vi "Assert Equal Type_Variant.vi"(4 "Execution time (s)":dbl=-1.0, 5 "Assert Only? (F)":bool, 6 "error code (1)":i32=1, 7 "Label":string, 8 "error in (no error)":errorcluster, 9 "Register with caller test (F)":bool, 10 "Actual":variant, 11 "Expected":variant) -> (0 "error out":errorcluster, 2 "Properties.Assert":refnum<class "Properties.Assert.lvclass">)   [LabVIEW 2013, in "Caraya.lvlib" / "Assert.lvclass"]
doc: "Generates an error if the input condition is not met.\n\nThis method compares the value of the inputs, irrespective of the type representation.\nAsserts TRUE if input values are equal.\nAsserts FALSE otherwise.\n\nex: Two integer inputs of equal value but of different type representation (U8 and I32) will assert TRUE."
uses:
  Assert.lvclass
  Properties.Assert/Properties.Assert.lvclass
  Properties/Properties.lvclass
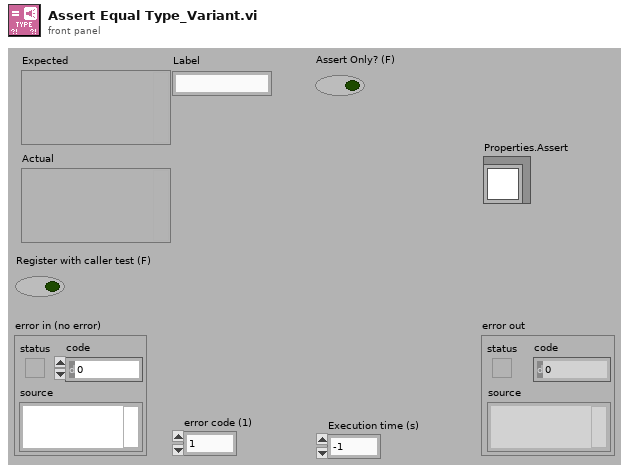
[diagram p1: front panel]
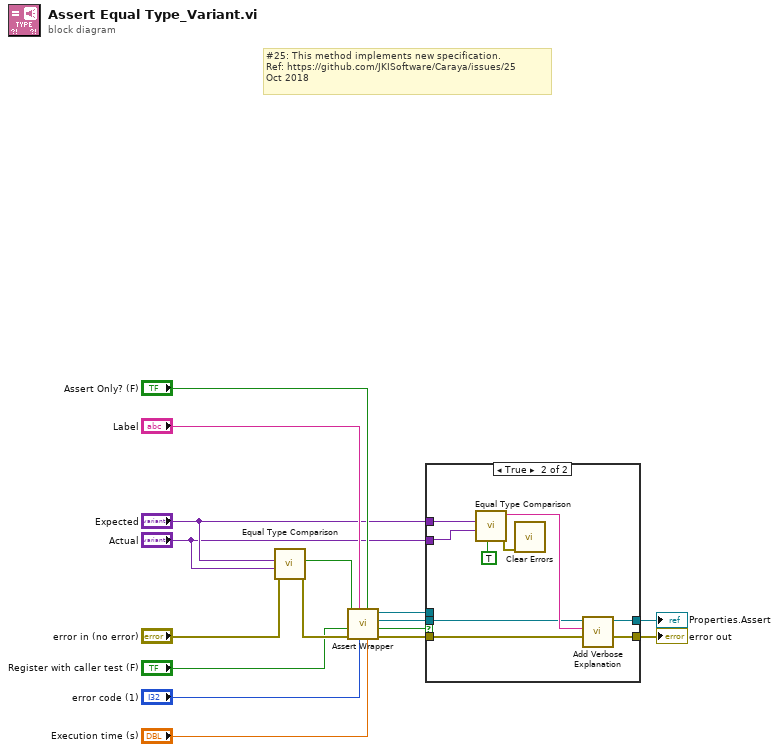
[diagram p0: block diagram]
diagram:
  # "#25: This method implements new specification.\nRef: https://github.com/JKISoftware/Caraya/issues/25\nOct 2018"
  n1 = call "Equal Type Comparison.vi"("error in (no error)"="error in (no error)", "Actual"="Actual", "Expected"="Expected") -> ("error out"=w13:errorcluster, "Equal Types?"=w12:bool)  [unwired: 6 in, 1 out]
  n2 = call "Assert Wrapper.vi"("Execution time (s)"="Execution time (s)", "Assert Only? (F)"="Assert Only? (F)", "error code (1)"="error code (1)", "Label"="Label", "error in (no error)"=w13, "Register with caller test (F)"="Register with caller test (F)", "Assert?"=w12) -> ("error out"=w9:errorcluster, "Verbose"=w5:bool, "Properties.Assert"=w2:refnum<class "Properties.Assert.lvclass">, "Assert out"=w3:refnum<class "Assert.lvclass">)  [unwired: 1 in]
  n3 = case shown="True" w5 {
    tunnel: [w18 w22] -> w10
    tunnel: w3 -> [_ _]
    tunnel: w9 -> [w18 w21]
    tunnel: "Expected" -> [_ w27]
    tunnel: "Actual" -> [_ w26]
    tunnel: w2 -> [w17 w20]
    tunnel: [w17 w19] -> w1
    frame False {
    }
    frame True {
      n4 = call "Equal Type Comparison.vi"("verbose? (F)"=TRUE, "Actual"=w26, "Expected"=w27) -> ("error out"=w24:errorcluster, "Verbose output"=w23:string)  [unwired: 6 in, 1 out]
      n5 = call <vilib>:"Clear Errors.vi"("error in (no error)"=w24) -> ()  [unwired: 6 in, 1 out]
      n6 = call "Add Verbose Explanation.vi"("error in (no error)"=w21, "Verbose Explanation"=w23, "Properties"=w20) -> ("error out"=w22:errorcluster, "Properties"=w19:refnum<class "Properties.Assert.lvclass">)  [unwired: 7 in]
    }
  }
  "error out" <- w10
  "Properties.Assert" <- w1
